vi "query TDF File List.vi"(8 "error in (no error)":errorcluster caption="에러 입력(에러 없음)", 11 "FSV-40N 입력":refnum<class "FSV-40N.lvclass">) -> (0 "error out":errorcluster caption="에러 출력", 2 "File List":string[](array[string]), 3 "FSV-40N 출력":refnum<class "FSV-40N.lvclass">)   [LabVIEW 2023, in "Spectrum Analyzer.lvlib" / "FSV-40N.lvclass"]
uses:
  FSV-40N.lvclass
  FSV-40N.lvclass/FSV-40N.ctl
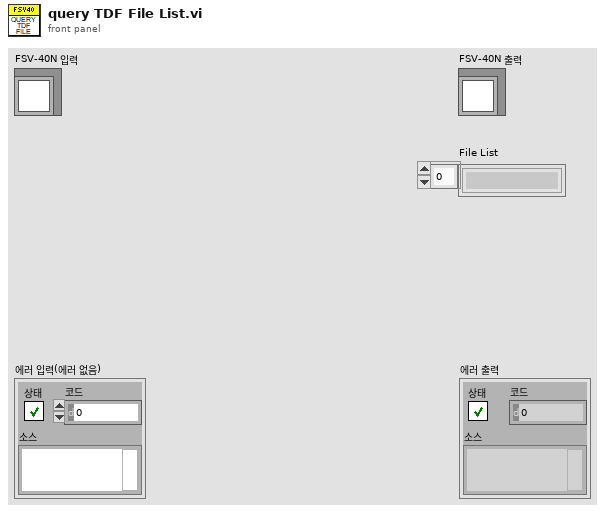
[diagram p1: front panel]
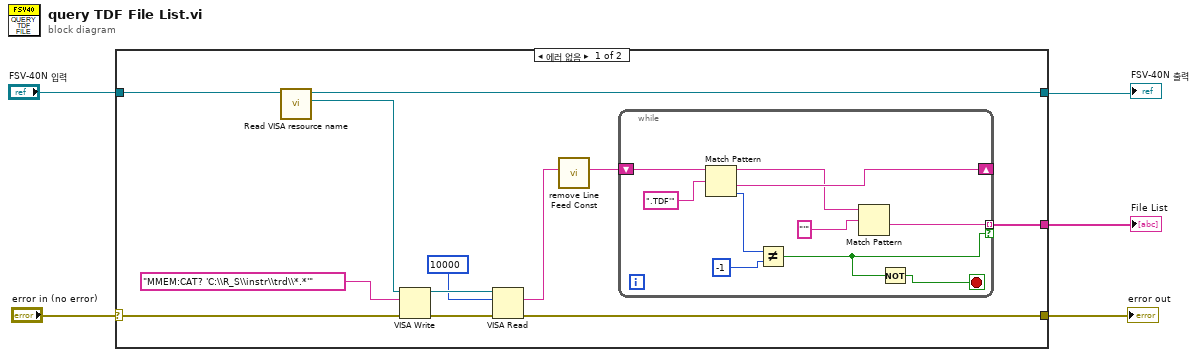
[diagram p0: block diagram]
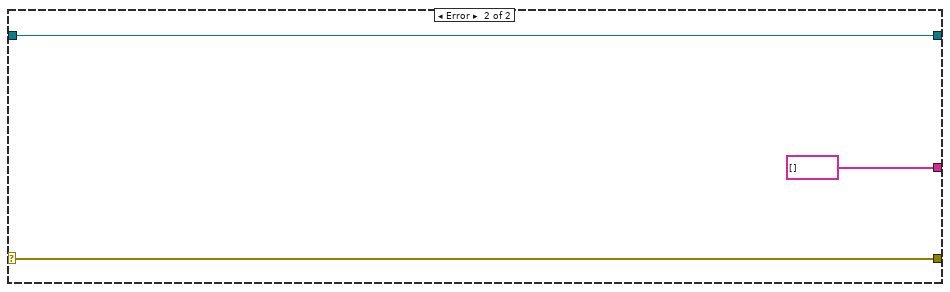
[diagram p2: hidden frame]
diagram:
  n1 = case shown="에러 없음" "error in (no error)" {
    selector: "error in (no error)" -> [w16 w29]
    tunnel: "FSV-40N 입력" -> [w17 w30]
    tunnel: [w9 w29] -> w3
    tunnel: [w8 w30] -> w2
    tunnel: [w6 string[] []] -> w1
    frame No Error {
      n2 = call "Read VISA resource name.vi"("FSV-40N in"=w17) -> ("VISA resource name"=w14:refnum<visa-resource-name>, "FSV-40N out"=w8:refnum<class "FSV-40N.lvclass">)  [unwired: 8 in, 1 out]
      n3 = VISA Write(VISA resource name=w14, write buffer="MMEM:CAT? 'C:\\R_S\\instr\\trd\\*.*'", error in (no error)=w16) -> (VISA resource name out=w12:refnum<visa-resource-name>, error out=w13:errorcluster)  [unwired: 1 out]
      n4 = VISA Read(VISA resource name=w12, byte count=u32 10000 ("바이트 카운트"), error in (no error)=w13) -> (read buffer=w10:string, error out=w9:errorcluster)  [unwired: 2 out]
      n5 = call "remove Line Feed Const.vi"("Input"=w10) -> ("Output"=w7:string)  [unwired: 10 in]
      n6 = while {
        shift-right: [w25] -> _
        shift-left: w7 -> [w26]
        tunnel: [w22] -> w6 mode=indexing if=w19
        stop <- w18 stop-if-true
        n7 = Match Pattern(string=w26, regular expression=".TDF'" ("정규식")) -> (before substring=w24:string, after substring=w25:string, offset past match=w21:i32)  [unwired: 1 in, 1 out]
        n8 = Not Equal?(x=w21, y=-1) -> (x != y?=w19:bool)
        n9 = Match Pattern(string=w24, regular expression="'" ("정규식")) -> (after substring=w22:string)  [unwired: 1 in, 3 out]
        n10 = Not(x=w19) -> (.not. x?=w18:bool)
      }
    }
    frame Error {
    }
  }
  "error out" <- w3
  "FSV-40N 출력" <- w2
  "File List" <- w1
